vi "Executor_Loop.vi"(8 "error in (no error)":errorcluster={"status"=FALSE, "code"=0, "source"="\"\""}, 10 "current time":i64=1000, 11 "StepContext":string="STEP_ACTIVE") -> (0 "error out":errorcluster={"status"=FALSE, "code"=0, "source"="\"\""}, 2 "status ok":bool, 3 "SequenceResult":string)   [LabVIEW 2026]
doc: "INTENT: Core sequence executor loop evaluating active step progress and endurance cycle counters."
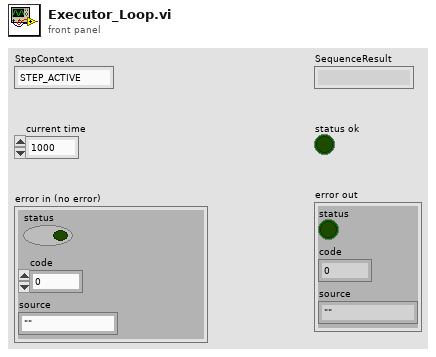
[diagram p1: front panel]
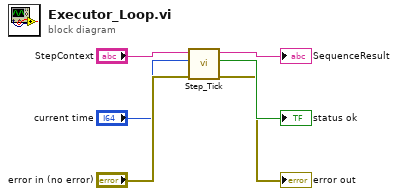
[diagram p0: block diagram]
diagram:
  n1 = call "Step_Tick.vi"("error in (no error)"="error in (no error)", "current time"="current time", "StepContext"="StepContext") -> ("error out"=→"error out":errorcluster, "status ok"=→"status ok":bool, "Updated StepContext and outgoing requests"=→"SequenceResult":string)  [unwired: 6 in]
